vi "Signal generator.vi"() -> ()   [LabVIEW 2018]
panel:
  in  "STOP":bool
  out "Waveform Graph":dynamicdata(graph)
  in  "Frequency":dbl(knob) scale=0.0..100.0
  in  "Amplitude":dbl(knob) scale=0.0..20.0
  in  "Enum":enum16{"Sine", "Triangle", "Sawtooth", "Square"}(ring)
  # "SIGNAL GENERTATOR"
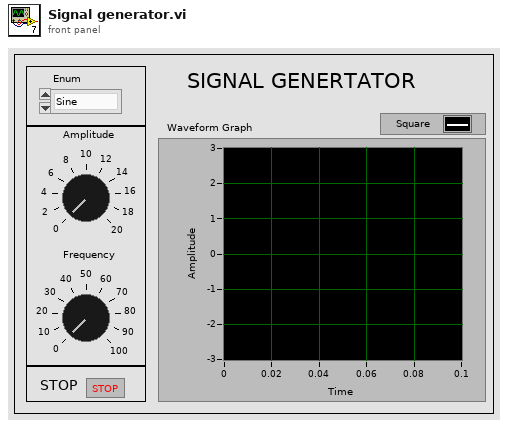
[diagram p1: front panel]
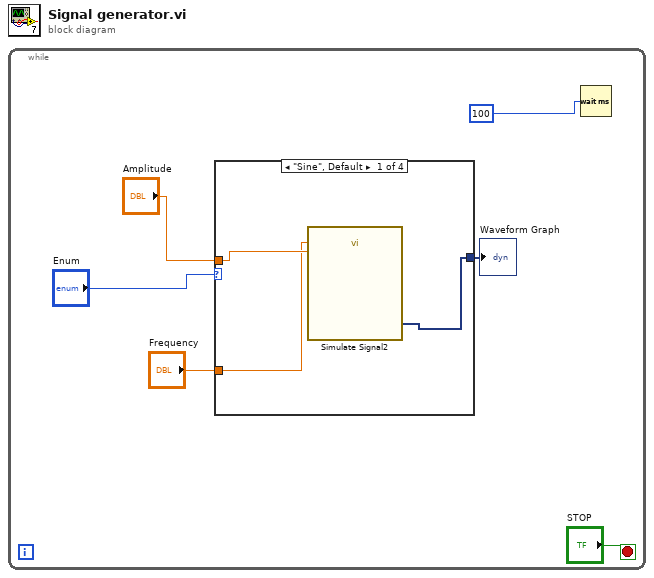
[diagram p0: block diagram]
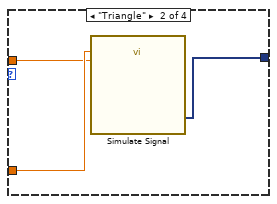
[diagram p2: hidden frame]
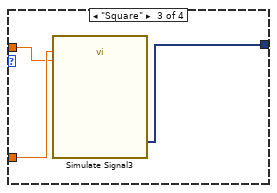
[diagram p3: hidden frame]
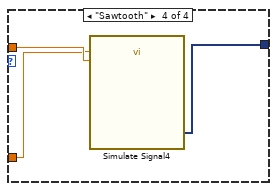
[diagram p4: hidden frame]
diagram:
  n1 = while {
    stop <- "STOP" stop-if-true
    n2 = case shown="\"Sine\", Default" "Enum" {
      tunnel: "Frequency" -> [w8 w12 w15 w17]
      tunnel: "Amplitude" -> [w9 w11 w14 w18]
      tunnel: [w7 w10 w13 w16] -> w3
      frame "Sine", Default {
        n3 = call "Simulate Signal2"("Frequency"=w8, "Amplitude"=w9) -> ("Sine"=w7:dynamicdata)  [unwired: 12 in, 1 out]
      }
      frame "Triangle" {
        n4 = call "Simulate Signal"("Frequency"=w12, "Amplitude"=w11) -> ("Triangle"=w10:dynamicdata)  [unwired: 12 in, 1 out]
      }
      frame "Square" {
        n5 = call "Simulate Signal3"("Frequency"=w15, "Amplitude"=w14) -> ("Square"=w13:dynamicdata)  [unwired: 12 in, 1 out]
      }
      frame "Sawtooth" {
        n6 = call "Simulate Signal4"("Frequency"=w17, "Amplitude"=w18) -> ("Sawtooth"=w16:dynamicdata)  [unwired: 12 in, 1 out]
      }
    }
    "Waveform Graph" <- w3
    n7 = Wait (ms)(milliseconds to wait=100) -> ()  [unwired: 1 out]
  }
